vi "Create (From State String Constant).vi"(8 "error in (no error)":errorcluster, 10 "State String Constant":refnum<vi>) -> (0 "error out":errorcluster, 1 "Structure Found in":refnum<vi>, 2 "Found JKI SMs?":bool, 3 "JKI SM out":refnum<class "JKI SM.lvclass">)   [LabVIEW 2020, in "JKI State Machine API.lvlib" / "JKI SM.lvclass"]
uses:
  JKI SM.lvclass
  JKI SM.lvclass/JKI SM.ctl
  JKI State Machine API.lvlib
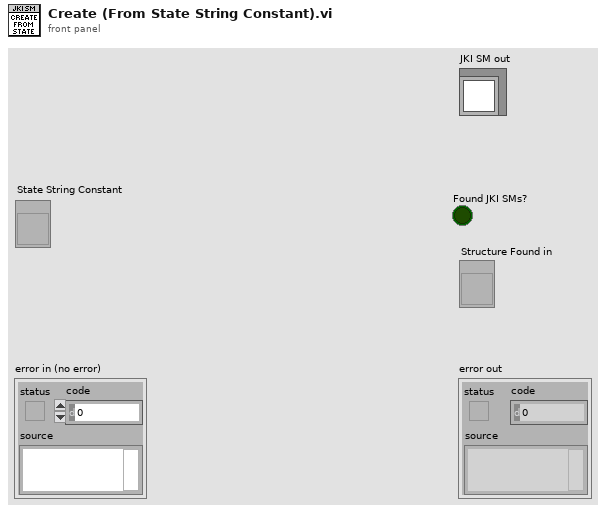
[diagram p1: front panel]
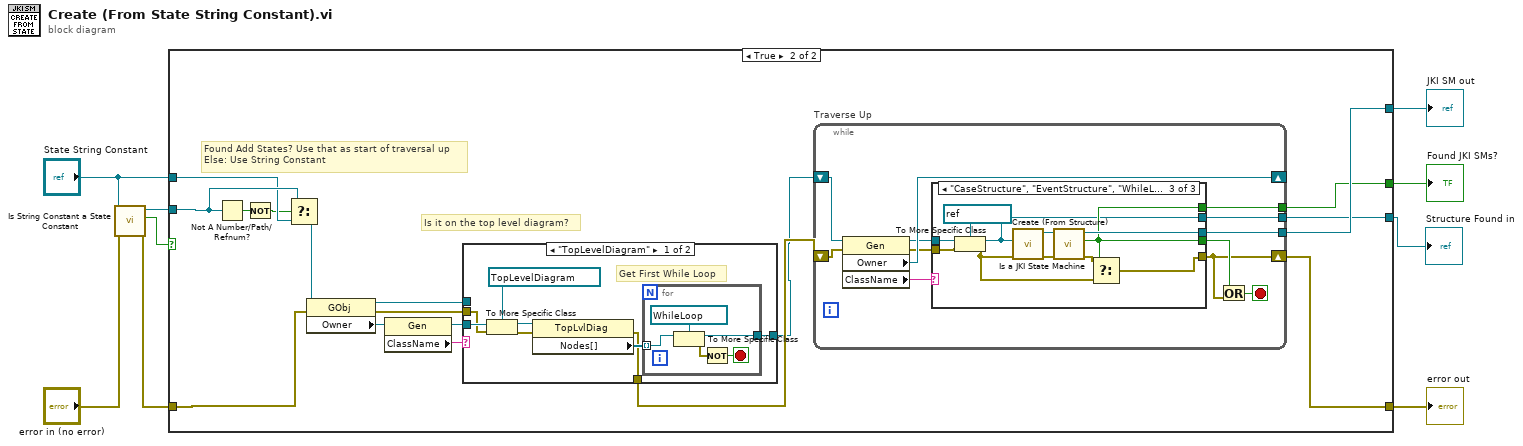
[diagram p0: block diagram]
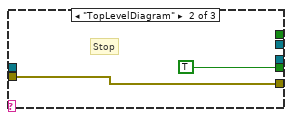
[diagram p5: hidden frame]
diagram:
  n1 = call "Is String Constant a State Constant.vi"("error in (no error)"="error in (no error)", "GObj Refnum"="State String Constant") -> ("error out"=w3:errorcluster, "Is States Constant"=w2:bool, "Add States to Queue"=w4:refnum<vi>)  [unwired: 7 in]
  n2 = case shown="True" w2 {
    tunnel: [w10 w26] -> w9
    tunnel: [_ w27] -> w8
    tunnel: "State String Constant" -> [_ w22]
    tunnel: [_ w25] -> w5
    tunnel: w4 -> [_ w24]
    tunnel: w3 -> [w10 w20]
    tunnel: [_ w19] -> w1
    frame False {
    }
    frame True {
      # "Is it on the top level diagram?"
      # "Found Add States? Use that as start of traversal up\nElse: Use String Constant"
      n3 = Not A Number/Path/Refnum?(number/path/refnum=w24) -> (NaN/Path/Refnum?=w18:bool)
      n4 = Not(x=w18) -> (.not. x?=w17:bool)
      n5 = Select(t=w24, s=w17, f=w22) -> (s? t:f=w15:refnum<vi>)
      n6 = property class="GObj"(reference=w15, error in=w20) -> (reference out=w16:refnum<vi>, error out=w14:errorcluster, "Owner"=w12:refnum<vi>)
      n7 = property class="Gen"(reference=w12) -> (reference out=w11:refnum<vi>, "ClassName"=w13:string)  [unwired: 1 in, 1 out]
      n8 = case shown="\"TopLevelDiagram\"" w13 {
        tunnel: w16 -> [_ w42]
        tunnel: w11 -> [w35 _]
        tunnel: [w31 w42] -> w21
        tunnel: w14 -> [w29 w41]
        tunnel: [w28 w41] -> w23
        frame "TopLevelDiagram" {
          # "Get First While Loop"
          n9 = To More Specific Class(target class=refnum<vi> refnum ("Owner"), reference=w35, error in=w29) -> (specific class reference=w33:refnum<vi>, error out=w30:errorcluster)
          n10 = property class="TopLvlDiag"(reference=w33, error in=w30) -> (error out=w28:errorcluster, "Nodes[]"=w32:refnum<vi>[])  [unwired: 1 out]
          n11 = for {
            tunnel: w32 -> [w40] mode=indexing
            tunnel: [w37] -> w31
            stop <- w36 stop-if-true
            n12 = To More Specific Class(target class=refnum<vi> refnum ("Owner"), reference=w40) -> (specific class reference=w37:refnum<vi>, error out=w38:errorcluster)  [unwired: 1 in]
            n13 = Not(x=w38) -> (.not. x?=w36:bool)
          }
        }
        frame Default {
        }
      }
      n14 = while "Traverse Up" {
        shift-right: [w54] -> _
        shift-left: w21 -> [w53]
        shift-right: [w45] -> w26
        shift-left: w23 -> [w49]
        tunnel: [w48] -> w27
        tunnel: [w44] -> w25
        tunnel: [w43] -> w19
        stop <- w47 stop-if-true
        n15 = property class="Gen"(reference=w53, error in=w49) -> (reference out=w51:refnum<vi>, error out=w50:errorcluster, "Owner"=w54:refnum<vi>, "ClassName"=w52:string)
        n16 = case shown="\"CaseStructure\", \"EventStructure\", \"WhileLoop\"" w52 {
          tunnel: w51 -> [_ _ w68]
          tunnel: [w55 w57 w60] -> w45
          tunnel: w50 -> [w55 w57 w66]
          tunnel: [_ _ w64] -> w48
          tunnel: [_ TRUE ("Is a JKI State Machine") w59] -> w46
          tunnel: [_ _ w59] -> w44
          tunnel: [_ _ w58] -> w43
          frame Default {
          }
          frame "TopLevelDiagram" {
            # "Stop"
          }
          frame "CaseStructure", "EventStructure", "WhileLoop" {
            n17 = To More Specific Class(target class=refnum<vi> refnum ("Structure"), reference=w68, error in=w66) -> (specific class reference=w58:refnum<vi>, error out=w61:errorcluster)
            n18 = call "Create (From Structure).vi"("error in (no error)"=w61, "Structure"=w58) -> ("error out"=w63:errorcluster, "JKI SM out"=w65:refnum<class "JKI SM.lvclass">)  [unwired: 8 in]
            n19 = call "Is a JKI State Machine.vi"("error in (no error)"=w63, "JKI SM in"=w65) -> ("error out"=w62:errorcluster, "Is a JKI State Machine"=w59:bool, "JKI SM out"=w64:refnum<class "JKI SM.lvclass">)  [unwired: 7 in]
            n20 = Select(t=w62, s=w59, f=w61) -> (s? t:f=w60:errorcluster)
          }
        }
        n21 = Or(x=w46, y=w45) -> (x .or. y?=w47:bool)
      }
    }
  }
  "error out" <- w9
  "JKI SM out" <- w8
  "Found JKI SMs?" <- w5
  "Structure Found in" <- w1
